vi "libssh2_userauth_publickey_frommemory.vi"(5 "private key data":string, 7 "public key data":string, 8 "error in (no error)":errorcluster, 9 "passphrase":string, 10 "username":string, 11 "session":T1) -> (0 "error out":errorcluster)   [LabVIEW 2017, in "libssh2.lvlib"]
doc: "Authenticate a session using a private and public key from memory."
uses:
  libssh2.lvlib
  Session Refnum.ctl
  Not A Session.vi
  <vilib>/Utility/error.llb/Error Cluster From Error Code.vi
  Global Settings.vi
  Read Session Refnum.vi
  <vilib>/Utility/semaphor.llb/Acquire Semaphore.vi
  <vilib>/Utility/semaphor.llb/Release Semaphore.vi
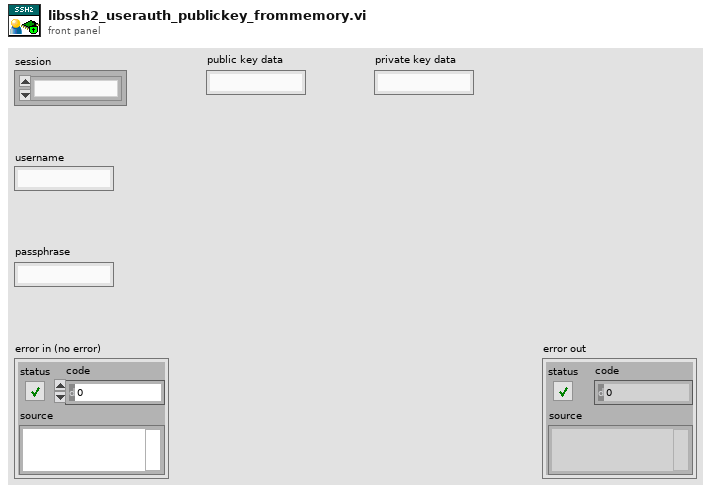
[diagram p1: front panel]
types:
  T1 = typedef "libssh2.lvlib/Session Refnum.ctl" = refnum<k1>
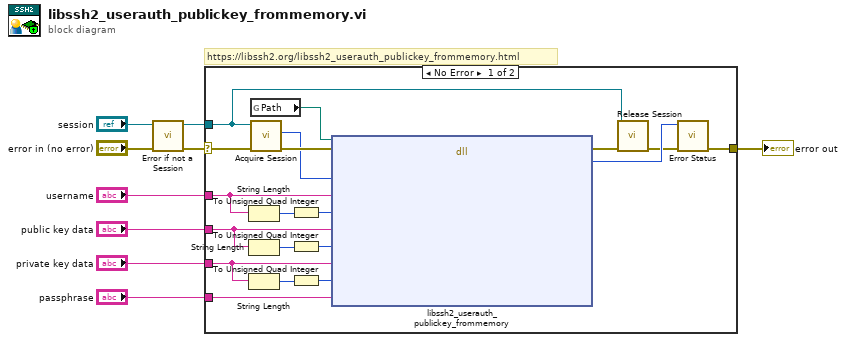
[diagram p0: block diagram]
diagram:
  # "https://libssh2.org/libssh2_userauth_publickey_frommemory.html"
  n1 = call "Error if not a Session.vi"("error in (no error)"="error in (no error)", "session"="session") -> ("error out"=w6:errorcluster, "session out"=w4:T1)  [unwired: 8 in]
  n2 = case shown="No Error" w6 {
    selector: w6 -> [w27 w29]
    tunnel: "username" -> [w28 _]
    tunnel: [w26 w29] -> w8
    tunnel: w4 -> [w10 _]
    tunnel: "public key data" -> [w12 _]
    tunnel: "private key data" -> [w13 _]
    tunnel: "passphrase" -> [w18 _]
    frame No Error {
      n3 = String Length(string=w28) -> (length=w23:i32)
      n4 = String Length(string=w12) -> (length=w17:i32)
      n5 = String Length(string=w13) -> (length=w16:i32)
      n6 = global read "Global Settings.vi" "Path"() -> (w20:path)
      n7 = call "Acquire Session.vi"("error in (no error)"=w27, "session"=w10) -> ("error out"=w22:errorcluster, "LIBSSH2_SESSION*"=w21:u64)  [unwired: 7 in, 1 out]
      n8 = To Unsigned Quad Integer(1:w23) -> (0:w25:u64)
      n9 = To Unsigned Quad Integer(1:w17) -> (0:w14:u64)
      n10 = To Unsigned Quad Integer(1:w16) -> (0:w15:u64)
      n11 = dll-call lib="?" fn="libssh2_userauth_publickey_frommemory"(path in=w20, error in=w22, "session"=w21, "username"=w28, "username_len"=w25, "publickeyfiledata"=w12, "publickeyfiledata_len"=w14, "privatekeyfiledata"=w13, "privatekeyfiledata_len"=w15, "passphrase"=w18) -> (error out=w24:errorcluster, "return value"=w19:i32)  [unwired: 9 in, 1 out]
      n12 = call "Release Session.vi"("error in (no error)"=w24, "session"=w10) -> ("error out"=w11:errorcluster)  [unwired: 9 in]
      n13 = call "Error Status.vi"("error in (no error)"=w11, "return value"=w19) -> ("error out"=w26:errorcluster)  [unwired: 8 in, 1 out]
    }
    frame Error {
    }
  }
  "error out" <- w8
